vi "Handle Zoom Event.vi"(6 "Coords":T1, 8 "error in":errorcluster, 9 "Zoom History":cluster{"X":sgl, "Y":sgl}[](array[cluster]), 10 "Zoom Type":enum32{"Zoom In", "Zoom Out"}(ring)=enum."Zoom Out", 11 "BigMAQ in":refnum<class "BigMAQ.lvclass">) -> (0 "error out":errorcluster, 1 "Discard?":bool, 2 "Zoom Out?":bool, 3 "BigMAQ out":refnum<class "BigMAQ.lvclass">)   [LabVIEW 2019, in "BigMAQ.lvclass"]
uses:
  BigMAQ.lvclass
  <vilib>/Utility/miscctls.llb/LVPoint32TypeDef.ctl
  BigMAQ.lvclass/BigMAQ.ctl
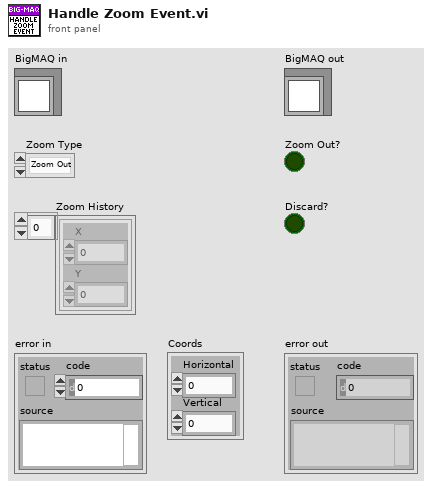
[diagram p1: front panel]
types:
  T1 = typedef "LVPoint32TypeDef.ctl" = cluster{"Horizontal":i32, "Vertical":i32}
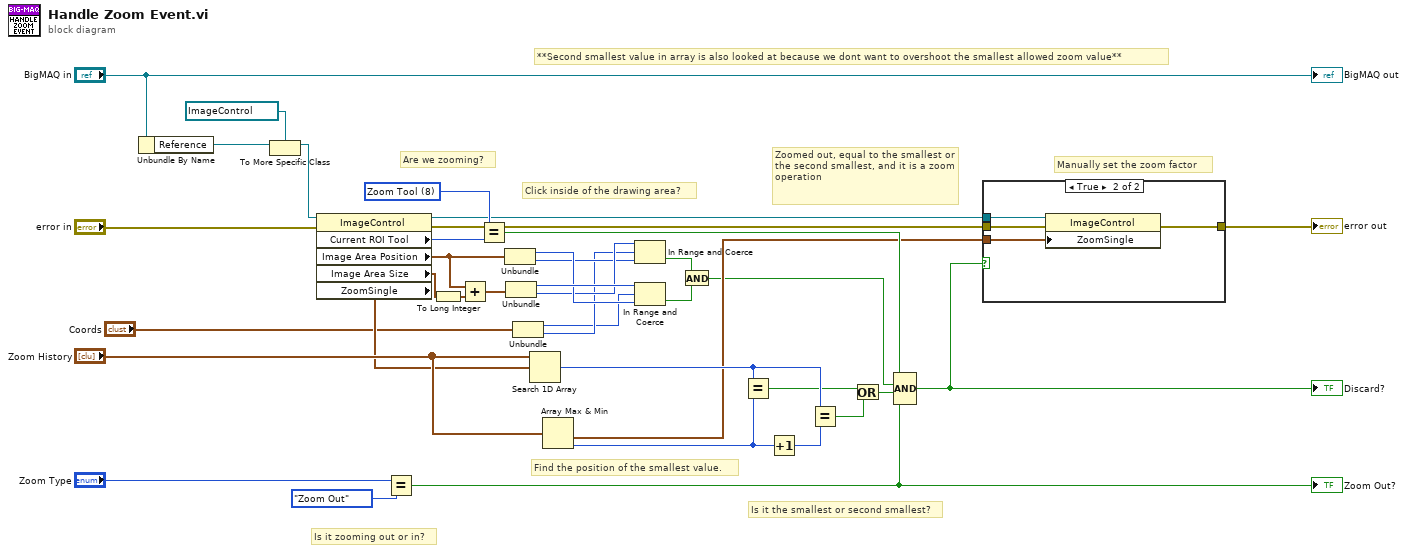
[diagram p0: block diagram]
diagram:
  w37 = u32 8 items=["Zoom Tool"=8, "Selection Tool"=0, "Pan Tool"=9, "Point Tool"=1, "Line Tool"=2, "Rectangle Tool"=3, "Rotated Rectangle Tool"=12, "Polyline Tool"=10, "Polygon Tool"=5, "Freehand Tool"=11, "Closed Freehand Tool"=6, "Ellipse Tool"=4, "Annulus Tool"=7] ("Current ROI Tool")
  # "Manually set the zoom factor"
  # "Are we zooming?"
  # "**Second smallest value in array is also looked at because we dont want to overshoot the smallest allowed zoom value**"
  # "Is it the smallest or second smallest?"
  # "Find the position of the smallest value."
  # "Is it zooming out or in?"
  # "Click inside of the drawing area?"
  # "Zoomed out, equal to the smallest or the second smallest, and it is a zoom operation"
  n1 = Unbundle By Name("BigMAQ in") -> ("Reference"=w1:refnum<vi>)
  n2 = To More Specific Class(target class=refnum<vi> refnum ("reference"), reference=w1) -> (specific class reference=w2:refnum<vi>)  [unwired: 1 in, 1 out]
  n3 = property class="ImageControl"(reference=w2, error in="error in") -> (reference out=w24:refnum<vi>, error out=w21:errorcluster, "Current ROI Tool"=w36:u32, "Image Area Position"=w14:cluster{"Left":i32, "Top":i32}, "Image Area Size"=w17:cluster{"Width":u32, "Height":u32}, "ZoomSingle"=w16:cluster{"X":sgl, "Y":sgl})
  n4 = Equal?(x="Zoom Type", y=enum32{"Zoom In", "Zoom Out"}."Zoom Out" ("Zoom Type")) -> (x = y?=w28:bool)
  "Zoom Out?" <- w28
  n5 = To Long Integer(number=w17) -> (32bit integer=w5:cluster{"Width":i32, "Height":i32})
  n6 = Add(x=w14, y=w5) -> (x+y=w15:cluster{i32, i32})
  n7 = Equal?(x=w37, y=w36) -> (x = y?=w26:bool)
  n8 = Unbundle(w14) -> ("Left"=w12:i32, "Top"=w10:i32)
  n9 = Unbundle(w15) -> (w13:i32, w11:i32)
  n10 = Unbundle("Coords") -> ("Horizontal"=w4:i32, "Vertical"=w8:i32)
  n11 = Search 1D Array(1D array="Zoom History", element=w16) -> (index of element=w30:i32)  [unwired: 1 in]
  n12 = Array Max & Min(array="Zoom History") -> (min value=w23:cluster{"X":sgl, "Y":sgl}, min index (indices)=w32:i32)  [unwired: 2 out]
  n13 = In Range and Coerce(upper limit=w11, x=w8, lower limit=w10) -> (In Range?=w7:bool)  [unwired: 1 out]
  n14 = In Range and Coerce(upper limit=w13, x=w4, lower limit=w12) -> (In Range?=w6:bool)  [unwired: 1 out]
  n15 = And(x=w7, y=w6) -> (x .and. y?=w3:bool)
  n16 = Equal?(x=w30, y=w32) -> (x = y?=w29:bool)
  n17 = Increment(x=w32) -> (x+1=w31:i32)
  n18 = Equal?(x=w30, y=w31) -> (x = y?=w22:bool)
  n19 = Or(x=w29, y=w22) -> (x .or. y?=w27:bool)
  n20 = Compound Arithmetic op=AND(w26, w3, w27, w28) -> (w25:bool)
  "Discard?" <- w25
  n21 = case shown="True" w25 {
    tunnel: w24 -> [_ w43]
    tunnel: w23 -> [_ w42]
    tunnel: [w39 w41] -> w19
    tunnel: w21 -> [w39 w40]
    frame False {
    }
    frame True {
      n22 = property class="ImageControl"(reference=w43, error in=w40, "ZoomSingle"=w42) -> (error out=w41:errorcluster)  [unwired: 1 out]
    }
  }
  "error out" <- w19
  "BigMAQ out" <- "BigMAQ in"
